vi "test--Hue--361degrees.vi"(11 "Test Case In":refnum<class "HSL Hue Wrap.lvclass">) -> (0 "error out":errorcluster, 3 "Test Case Out":refnum<class "HSL Hue Wrap.lvclass">)   [LabVIEW 2021, in "HSL Hue Wrap.lvclass"]
uses:
  HSL Hue Wrap.lvclass
  C:/Program Files/National Instruments/LabVIEW 2026/vi.lib/Astemes/LUnit/Test Case.lvclass
  <vilib>/Astemes/LUnit/Test Case.lvclass/Test Case.ctl
  HSL Hue Wrap.lvclass/HSL Hue Wrap.ctl
  4993e8ee-a06a-463a-9684-69129f64d5ce.vi
  src/Material SubVIs/Material SubVIs.lvlib
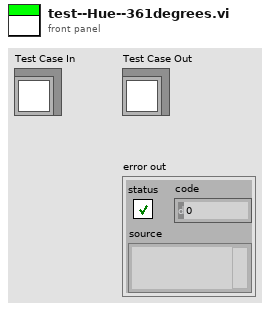
[diagram p1: front panel]
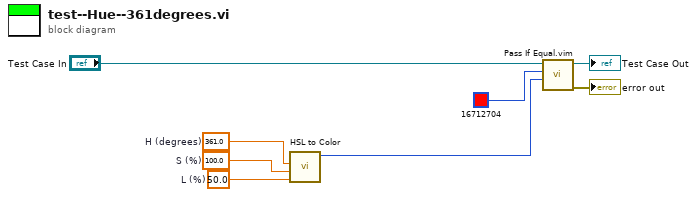
[diagram p0: block diagram]
diagram:
  w3 = 361.0  # H (degrees)
  w4 = 100.0  # S (%)
  w5 = 50.0  # L (%)
  n1 = call "HSL to Color.vi"("L (%)"=w5, "S (%)"=w4, "H (degrees)"=w3) -> ("Color out"=w2:u32)  [unwired: 5 in, 3 out]
  n2 = call "Pass If Equal.vim"("Actual"=w2, "Expected"=u32 16712704, "LUnit Test Case In"="Test Case In") -> ("error out"=→"error out":errorcluster, "LUnit Test Case Out"=→"Test Case Out":refnum<class "HSL Hue Wrap.lvclass">)  [unwired: 7 in]
